vi "plcm3GetValue.vi"(6 "Measurement Type":u32(ring) items=["OFF", "1mV range (1mV/A)", "10mV range (10mV/A)", "100mV range (100mV/A)", "Voltage Input"], 7 "Channel":i32, 8 "error in (no error)":errorcluster, 11 "handle in":i16) -> (0 "error out":errorcluster, 1 "PICO_STATUS out":T1, 2 "Channel Data":dbl, 3 "handle out":i16)   [LabVIEW 2010]
doc: "Calls UsbPt104GetValue for single channel, returns single value."
uses:
  plcm3.dll
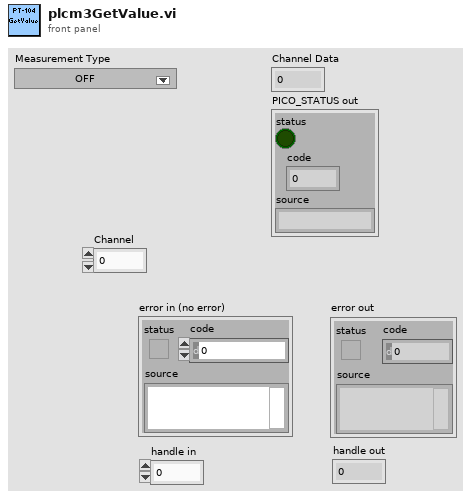
[diagram p1: front panel]
types:
  T1 = cluster{"status":bool, "code":u32, "source":string}
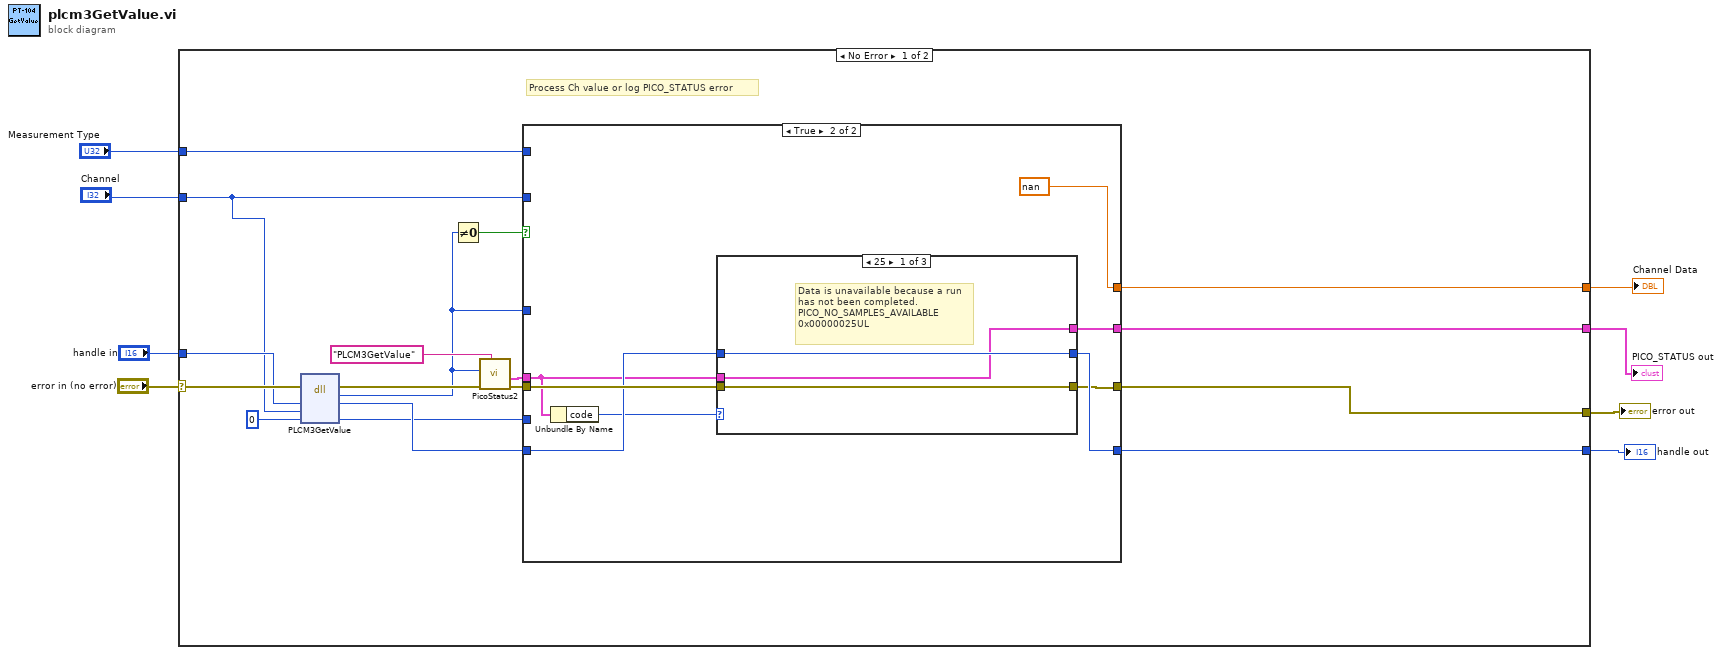
[diagram p0: block diagram]
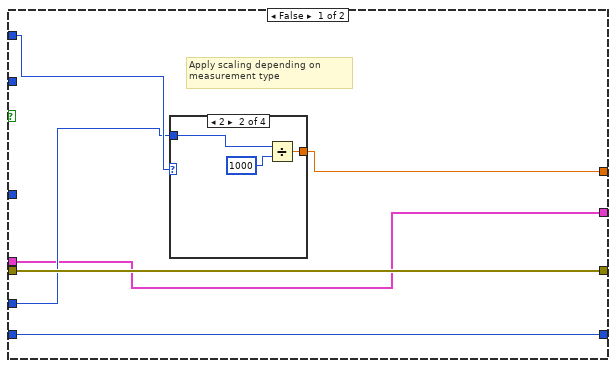
[diagram p2: hidden frame]
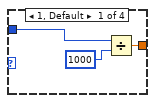
[diagram p3: hidden frame]
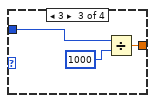
[diagram p4: hidden frame]
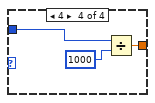
[diagram p5: hidden frame]
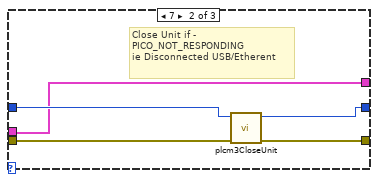
[diagram p6: hidden frame]
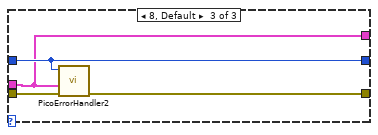
[diagram p7: hidden frame]
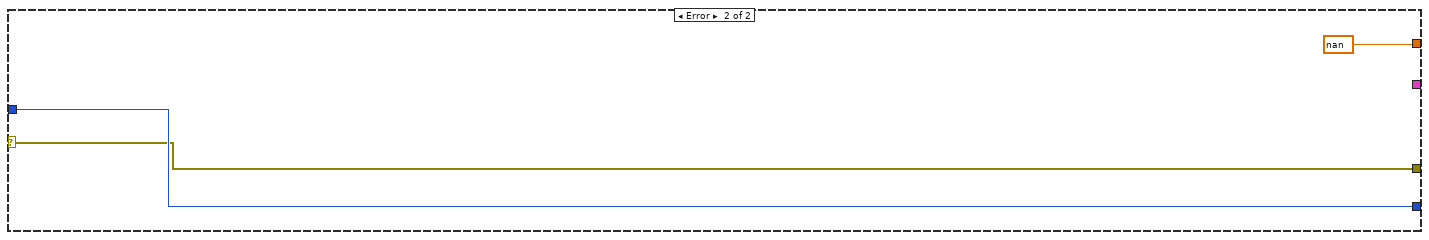
[diagram p8: hidden frame]
diagram:
  n1 = case shown="No Error" "error in (no error)" {
    selector: "error in (no error)" -> [w22 w65]
    tunnel: "handle in" -> [w21 w66]
    tunnel: [w23 w66] -> w8
    tunnel: [w24 w65] -> w7
    tunnel: "Channel" -> [w15 _]
    tunnel: "Measurement Type" -> [w17 _]
    tunnel: [w16 nan] -> w2
    tunnel: [w9 _] -> w1
    frame No Error {
      # "Process Ch value or log PICO_STATUS error"
      n2 = dll-call lib="PLCM3.dll" fn="PLCM3GetValue"(error in=w22, "handle"=w21, "channel"=w15, "value"=0) -> (error out=w13:errorcluster, "PICO_STATUS"=w12:u32, "handle"=w20:i16, "value"=w19:i32)  [unwired: 3 in, 1 out]
      n3 = Not Equal To 0?(x=w12) -> (x != 0?=w25:bool)
      n4 = call "PicoStatus2.vi"("PICO source"="PLCM3GetValue" ("source"), "Error in"=w13, "PICO STATUS"=w12) -> ("error out"=w11:errorcluster, "PICO_STATUS out"=w10:T1)  [unwired: 5 in]
      n5 = case shown="True" w25 {
        tunnel: w11 -> [w30 w51]
        tunnel: w15 -> [_ _]
        tunnel: w20 -> [w31 w47]
        tunnel: [w31 w50] -> w23
        tunnel: [w30 w49] -> w24
        tunnel: w12 -> [_ _]
        tunnel: [w27 nan] -> w16
        tunnel: w19 -> [w28 _]
        tunnel: w17 -> [w29 _]
        tunnel: w10 -> [w26 w45]
        tunnel: [w26 w44] -> w9
        frame False {
          # "Apply scaling depending on \nmeasurement type"
          n6 = case shown="2" w29 {
            tunnel: w28 -> [w33 w36 w39 w42]
            tunnel: [w32 w35 w38 w41] -> w27
            frame 1, Default {
              n7 = Divide(x=w33, y=1000) -> (x/y=w32:dbl)
            }
            frame 2 {
              n8 = Divide(x=w36, y=1000) -> (x/y=w35:dbl)
            }
            frame 3 {
              n9 = Divide(x=w39, y=1000) -> (x/y=w38:dbl)
            }
            frame 4 {
              n10 = Divide(x=w42, y=1000) -> (x/y=w41:dbl)
            }
          }
        }
        frame True {
          n11 = Unbundle By Name(w45) -> ("code"=w46:u32)
          n12 = case shown="25" w46 {
            tunnel: w47 -> [w54 w56 w62]
            tunnel: w51 -> [w53 w59 w63]
            tunnel: [w54 w57 w62] -> w50
            tunnel: [w53 w58 w61] -> w49
            tunnel: w45 -> [w52 w55 w60]
            tunnel: [w52 w55 w60] -> w44
            frame 37 {
              # "Data is unavailable because a run\nhas not been completed.\nPICO_NO_SAMPLES_AVAILABLE \n0x00000025UL"
            }
            frame 7 {
              # "Close Unit if -\nPICO_NOT_RESPONDING\nie Disconnected USB/Etherent"
              n13 = call "plcm3CloseUnit.vi"("error in (no error)"=w59, "handle in"=w56) -> ("error out"=w58:errorcluster, "handle out"=w57:i16)  [unwired: 8 in]
            }
            frame 8, Default {
              n14 = call "PicoErrorHandler2.vi"("error in (no error)"=w63, "PICO_STATUS in"=w60, "handle In"=w62) -> ("error out"=w61:errorcluster)  [unwired: 8 in]
            }
          }
        }
      }
    }
    frame Error {
    }
  }
  "error out" <- w7
  "handle out" <- w8
  "Channel Data" <- w2
  "PICO_STATUS out" <- w1
